vi "Descriptor_ExtractElements.vi"(10 "Descriptor":T1) -> (0 "concatenated element descriptors":i16[](array[numeric]), 1 "Nb elements":i32, 2 "Descriptor Elements":T1[](array[typedef]))   [LabVIEW 2013, in "OpenDescriptor.lvlib"]
uses:
  OpenDescriptor.lvlib
  OpenDescriptor -- cluster.ctl
  TypeDescriptor_GetPString.vi
  Conversions/OpenConvert.lvlib
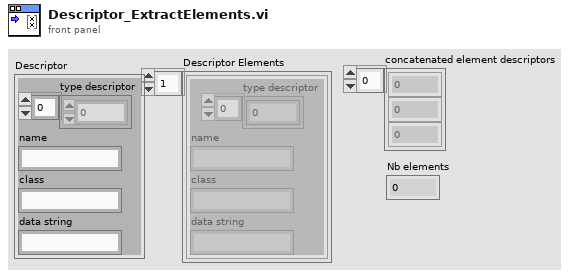
[diagram p1: front panel]
types:
  T1 = typedef "OpenDescriptor.lvlib/OpenDescriptor -- cluster.ctl" = cluster{"type descriptor":i16[], "name":string, "class":string, "data string":string}
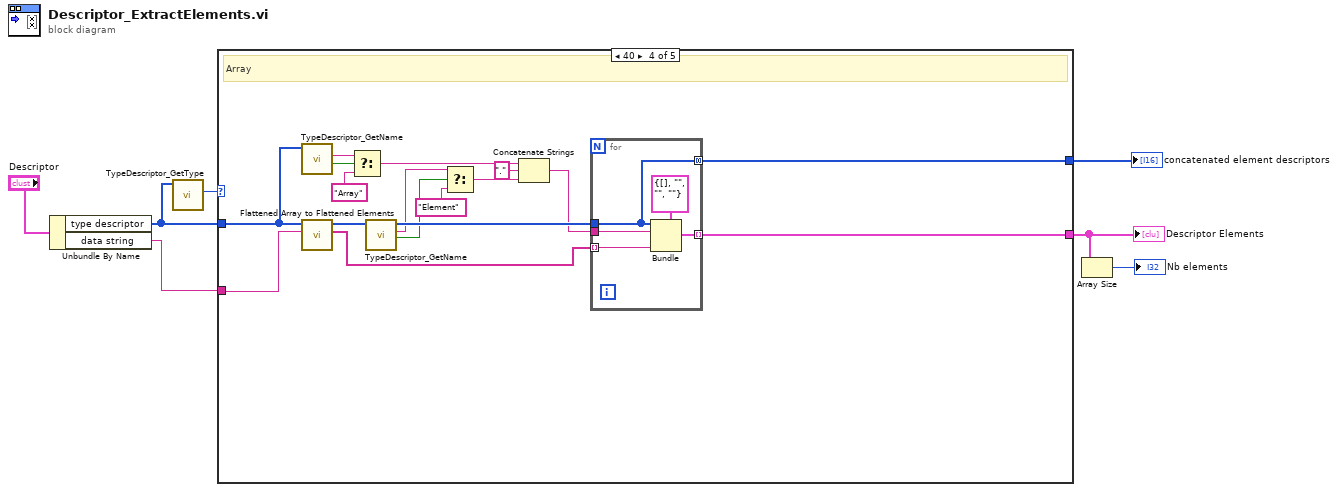
[diagram p0: block diagram]
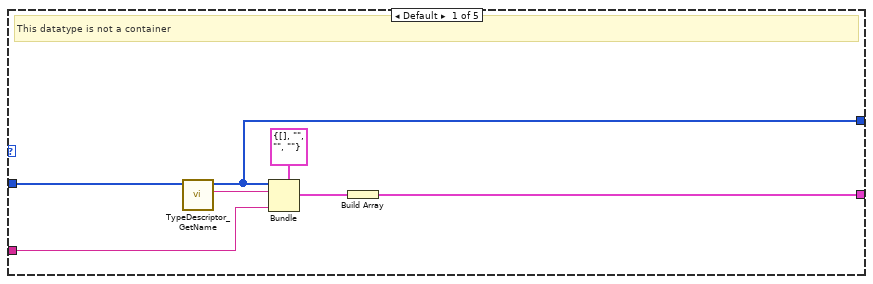
[diagram p2: hidden frame]
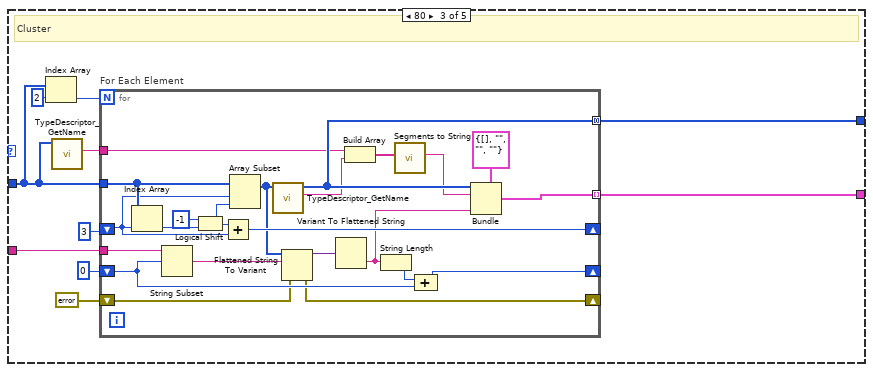
[diagram p4: hidden frame]
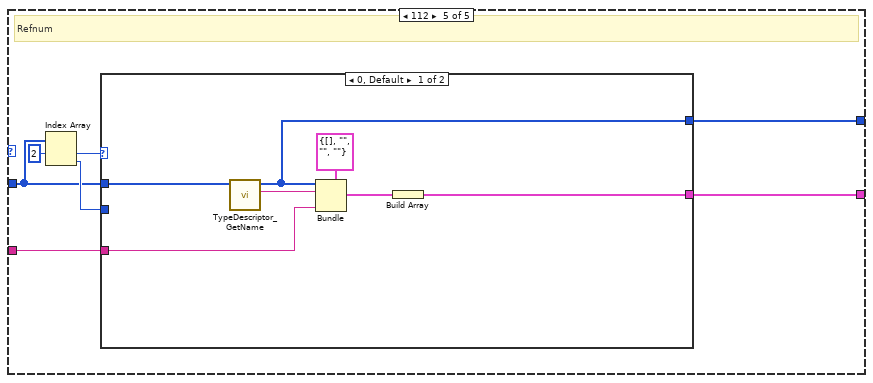
[diagram p5: hidden frame]
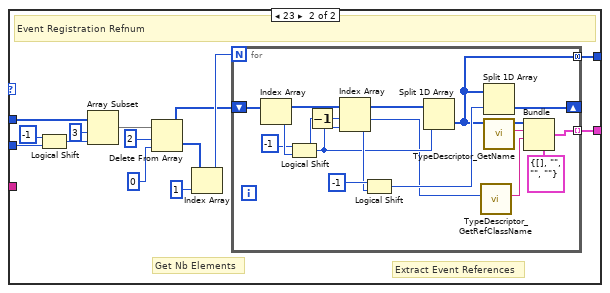
[diagram p6: hidden frame]
diagram:
  n1 = Unbundle By Name("Descriptor") -> ("type descriptor"=w2:i16[], "data string"=w1:string)
  n2 = call "TypeDescriptor_GetType.vi"("type descriptor"=w2) -> ("Type"=w3:u8)  [unwired: 9 in, 1 out]
  n3 = case shown="40" w3 {
    tunnel: [w10 _ w21 w61 w72] -> w7
    tunnel: w2 -> [w12 _ w16 w57 w73]
    tunnel: [w9 _ w20 w60 w71] -> w5
    tunnel: w1 -> [w8 _ w18 w58 w70]
    frame Default {
      # "This datatype is not a container"
      n4 = call "TypeDescriptor_GetName.vi"("type descriptor"=w12) -> ("name"=w14:string, "type descriptor dup"=w9:i16[])  [unwired: 8 in, 1 out]
      n5 = Bundle(cluster=T1 {"type descriptor"=[], "name"="", "class"="", "data string"=""} ("Descriptor Element"), "type descriptor"=w9, "name"=w14, "data string"=w8) -> (w11:T1)  [unwired: 1 in]
      n6 = Build Array(w11) -> (w10:T1[])
    }
    frame 0 {
      # "void"
    }
    frame 80 {
      # "Cluster"
      n7 = Index Array(array=w16, index=2) -> (element=w23:i16)
      n8 = call "TypeDescriptor_GetName.vi"("type descriptor"=w16) -> ("name"=w15:string)  [unwired: 8 in, 2 out]
      n9 = for "For Each Element" {
        N: w23 -> [_]
        tunnel: w16 -> [w44]
        shift-right: [w45] -> _
        shift-left: 3 ("index") -> [w43]
        tunnel: [w41] -> w21 mode=indexing
        tunnel: [w39] -> w20 mode=concatenating
        shift-right: [w32] -> _
        shift-left: 0 -> [w33]
        tunnel: w18 -> [w38]
        shift-right: [w29] -> _
        shift-left: errorcluster {"status"=FALSE, "code"=0, "source"=""} ("error out") -> [w30]
        tunnel: w15 -> [w28]
        n10 = Index Array(array=w44, index=w43) -> (element=w46:i16)
        n11 = String Subset(string=w38, offset (0)=w33) -> (substring=w36:string)  [unwired: 1 in]
        n12 = Logical Shift(y=i16 -1, x=w46) -> (x << y=w42:i16)
        n13 = Add(x=w42, y=w43) -> (x+y=w45:i32)
        n14 = Array Subset(array=w44, index=w43, length=w42) -> (w37:i16[])
        n15 = call "TypeDescriptor_GetName.vi"("type descriptor"=w37) -> ("name"=w26:string, "type descriptor dup"=w39:i16[])  [unwired: 8 in, 1 out]
        n16 = Flattened String To Variant(4:w30, 6:w36, 7:w37) -> (0:w29:errorcluster, 3:w35:variant)
        n17 = Variant To Flattened String(Variant=w35) -> (data string=w31:string)  [unwired: 1 out]
        n18 = Build Array(w28, w26) -> (w27:string[])
        n19 = String Length(string=w31) -> (length=w34:i32)
        n20 = call "Segments to String.vi"("Segments"=w27) -> ("String"=w25:string)  [unwired: 10 in]
        n21 = Compound Arithmetic op=ADD(w34, w33) -> (w32:i32)
        n22 = Bundle(cluster=T1 {"type descriptor"=[], "name"="", "class"="", "data string"=""} ("Descriptor Element"), "type descriptor"=w39, "name"=w25, "data string"=w31) -> (w41:T1)  [unwired: 1 in]
      }
    }
    frame 64 {
      # "Array"
      n23 = call "TypeDescriptor_GetName.vi"("type descriptor"=w57) -> ("found"=w55:bool, "name"=w54:string)  [unwired: 8 in, 1 out]
      n24 = call "Flattened Array to Flattened Elements.vi"("Flattened Array String"=w58, "Array Type Descriptor"=w57) -> ("Flattened Array Elements"=w56:string[], "Array Element Type Descriptor"=w59:i16[])  [unwired: 8 in]
      n25 = Select(t=w54, s=w55, f="Array" ("string")) -> (s? t:f=w52:string)
      n26 = call "TypeDescriptor_GetName.vi"("type descriptor"=w59) -> ("found"=w48:bool, "name"=w49:string, "type descriptor dup"=w64:i16[])  [unwired: 8 in]
      n27 = Select(t=w49, s=w48, f="Element" ("string")) -> (s? t:f=w50:string)
      n28 = Concatenate Strings(w52, "." ("string"), w50) -> (w62:string)
      n29 = for {
        tunnel: w56 -> [w65] mode=indexing
        tunnel: [w68] -> w61 mode=indexing
        tunnel: w64 -> [w66]
        tunnel: w62 -> [w67]
        tunnel: [w66] -> w60 mode=concatenating
        n30 = Bundle(cluster=T1 {"type descriptor"=[], "name"="", "class"="", "data string"=""} ("Descriptor Element"), "type descriptor"=w66, "name"=w67, "data string"=w65) -> (w68:T1)  [unwired: 1 in]
      }
    }
    frame 112 {
      # "Refnum"
      n31 = Index Array(array=w73, index #1=2 ("index")) -> (element #1=w75:i16, element #2=w74:i16)  [unwired: 1 in]
      n32 = case shown="0, Default" w75 {
        tunnel: w74 -> [_ w94]
        tunnel: w73 -> [w80 w97]
        tunnel: [w78 w85] -> w72
        tunnel: [w79 w84] -> w71
        tunnel: w70 -> [w77 _]
        frame 0, Default {
          n33 = call "TypeDescriptor_GetName.vi"("type descriptor"=w80) -> ("name"=w81:string, "type descriptor dup"=w79:i16[])  [unwired: 8 in, 1 out]
          n34 = Bundle(cluster=T1 {"type descriptor"=[], "name"="", "class"="", "data string"=""} ("Descriptor Element"), "type descriptor"=w79, "name"=w81, "data string"=w77) -> (w83:T1)  [unwired: 1 in]
          n35 = Build Array(w83) -> (w78:T1[])
        }
        frame 23 {
          # "Extract Event References"
          # "Get Nb Elements"
          # "Event Registration Refnum"
          n36 = Logical Shift(y=i16 -1, x=w94) -> (x << y=w93:i16)
          n37 = Array Subset(array=w97, index=3, length=w93) -> (w92:i16[])
          n38 = Delete From Array(array=w92, length=2 ("index"), index=0) -> (deleted portion=w90:i16[], array with subset deleted=w86:i16[])
          n39 = Index Array(array=w90, index=1) -> (element=w87:i16)
          n40 = for {
            N: w87 -> [_]
            shift-right: [w105] -> _
            shift-left: w86 -> [w108]
            tunnel: [w100] -> w85 mode=indexing
            tunnel: [w98] -> w84 mode=concatenating
            n41 = Index Array(array=w108) -> (element=w113:i16)  [unwired: 1 in]
            n42 = Logical Shift(y=i16 -1, x=w113) -> (x << y=w107:i16)
            n43 = Decrement(x=w107) -> (x-1=w109:i16)
            n44 = Index Array(array=w108, index #1=w109, index #2=w107) -> (element #1=w104:i16, element #2=w110:i16)
            n45 = Logical Shift(y=i16 -1, x=w110) -> (x << y=w106:i16)
            n46 = Split 1D Array(array=w108, index=w107) -> (second subarray=w98:i16[])  [unwired: 1 out]
            n47 = call "TypeDescriptor_GetRefClassName.vi"("Ref Class"=w104) -> ("Reference Class"=w102:string)  [unwired: 10 in]
            n48 = Split 1D Array(array=w98, index=w106) -> (second subarray=w105:i16[])  [unwired: 1 out]
            n49 = call "TypeDescriptor_GetName.vi"("type descriptor"=w98) -> ("name"=w101:string, "type descriptor dup"=w103:i16[])  [unwired: 8 in, 1 out]
            n50 = Bundle(cluster=T1 {"type descriptor"=[], "name"="", "class"="", "data string"=""} ("Descriptor Element"), "type descriptor"=w103, "name"=w101, "class"=w102) -> (w100:T1)  [unwired: 1 in]
          }
        }
      }
    }
  }
  "Descriptor Elements" <- w7
  "concatenated element descriptors" <- w5
  n51 = Array Size(array=w7) -> (size(s)=→"Nb elements":i32)
